vi "set Peak Excursion.vi"(8 "error in (no error)":errorcluster caption="에러 입력(에러 없음)", 10 "숫자형":dbl, 11 "Keysight 9020A 입력":refnum<class "Keysight 9020A.lvclass">) -> (0 "error out":errorcluster caption="에러 출력", 3 "Keysight 9020A 출력":refnum<class "Keysight 9020A.lvclass">)   [LabVIEW 2023, in "Spectrum Analyzer.lvlib" / "Keysight 9020A.lvclass"]
uses:
  Keysight 9020A.lvclass
  Keysight 9020A.lvclass/Keysight 9020A.ctl
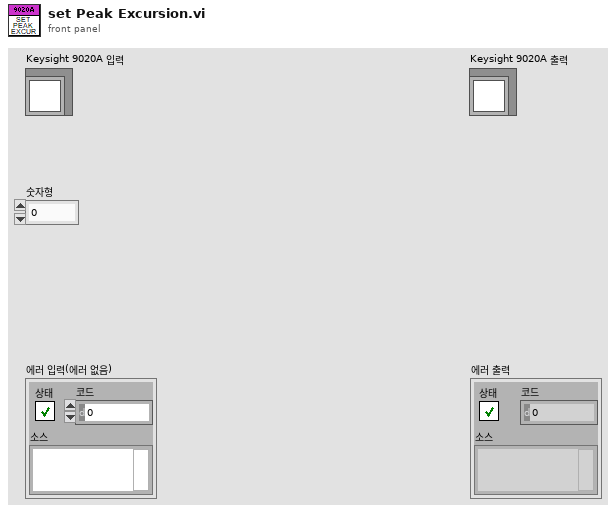
[diagram p1: front panel]
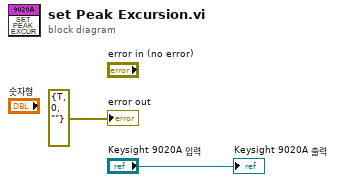
[diagram p0: block diagram]
diagram:
  "error out" <- errorcluster {"status"=TRUE, "code"=0, "source"=""} ("error out")
  "Keysight 9020A 출력" <- "Keysight 9020A 입력"
